vi "DualPump_ExplicitControl.vi"() -> ()   [LabVIEW 2025]
uses:
  <vilib>/Utility/error.llb/DialogType.ctl
  <vilib>/Instr/_visa.llb/VISA Configure Serial Port (Instr).vi
panel:
  out "Arduino Connected":bool
  in  "Arduino Connect Button":bool
  in  "Arduino Fluid Sensor COM Port":refnum<visa-resource-name>
  in  "quit":bool
  in  "Tab Control":enum32{"Control Interface", "Info and Help"}(tab)
  out "Pump #1 Filling":bool
  in  "Pump #1 Partial Fill Amount (µL)":dbl
  in  "Pump #2 Full Fill Button":bool
  in  "Pump #1 Partial Fill Button":bool
  out "Pump #2 Flavor Blasted Amount (µL)":dbl
  out "Pump #1 Flavor Blasted Amount (µL)":dbl
  in  "Pump #2 Start/Stop Button":bool
  in  "Pump #1 COM port":refnum<visa-resource-name>
  in  "Pump #1 flow rate (µL/min)":dbl=2000.0 format="%.3f"
  in  "Pump #2 COM port":refnum<visa-resource-name>
  in  "Pump #2 flow rate (µL/min)":dbl=5000.0 format="%.3f"
  in  "Pump #2 Flavor Blast Amount (µL)":dbl=75.0 format="%.3f"
  in  "Pump #1 syringe volume":dbl(ring)=28.75 items=["100 uL"=1.44, "1 mL"=4.75, "3 mL"=9.8, "5 mL"=11.83, "15 mL"=18.034, "20 mL"=19.304, "50 mL"=28.75]
  in  "Pump #2 syringe volume":dbl(ring)=28.75 items=["100 uL"=1.44, "1 mL"=4.75, "3 mL"=9.8, "5 mL"=11.83, "15 mL"=18.034, "20 mL"=19.304, "50 mL"=28.75]
  out "Pump #2 Flowing":bool
  in  "Pump 1 Connect":bool
  in  "Pump 2 Connect":bool
  out "Pump 2 Connected":bool
  out "Pump 1 Connected":bool
  in  "Pump #1 Flavor Blast Amount (µL)":dbl=200.0
  in  "Pump #1 Flavor Blast Button":bool
  out "Pump #1 Amount Remaining (µL)":dbl
  in  "Pump #1 Start/Stop Button":bool
  out "Pump #1 Flowing":bool
  out "Pump #2 Amount Remaining (µL)":dbl
  in  "Pump #2 Flavor Blast Button":bool
  in  "Pump #2 Partial Fill Button":bool
  in  "Pump #2 Partial Fill Amount (µL)":dbl
  in  "Pump #1 Full Fill Button":bool
  out "Pump #2 Filling":bool
  out "Interface Locked":bool
  # "1. Set Communication"
  # "Pump #1"
  # "Pump #2"
  # "This program is designed to only control the two New Era Syringe Pumps on-site in the Varro laboratory. It can be generalized for other use by adjusting the hard-coded \"firmware\" variables to match any pump.\n\nFull Fill will fill the syringe up to its maximum volume, specified by the chosen syringe volume. Partial Fill will fill the syringe up to the lesser of the chosen volume or the maximum volume.\n\nPumps flow continuously when Start is pressed. The pump will blast a specified amount at its flowrate setpoint when Blast It! is pressed.\n\nFilling and flavor blasting will block the interface, which will be indicated in the upper-right corner."
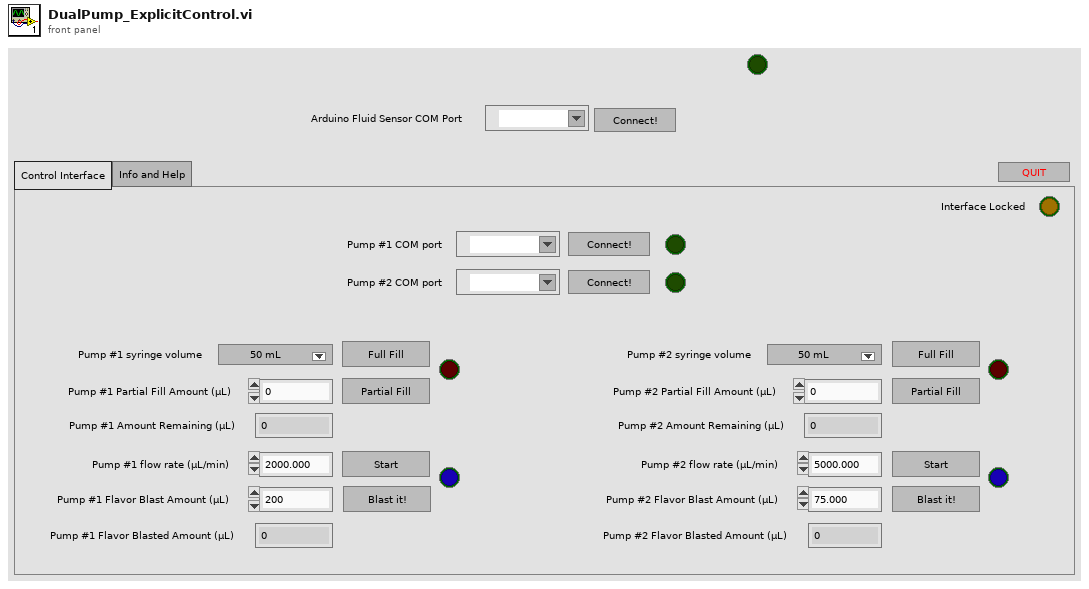
[diagram p1: front panel]
types:
  T1 = cluster{"0=off\n1=on":u16, "Numbers of beeps\n0=continuously":dbl}
  T2 = typedef "DialogType.ctl" = u16
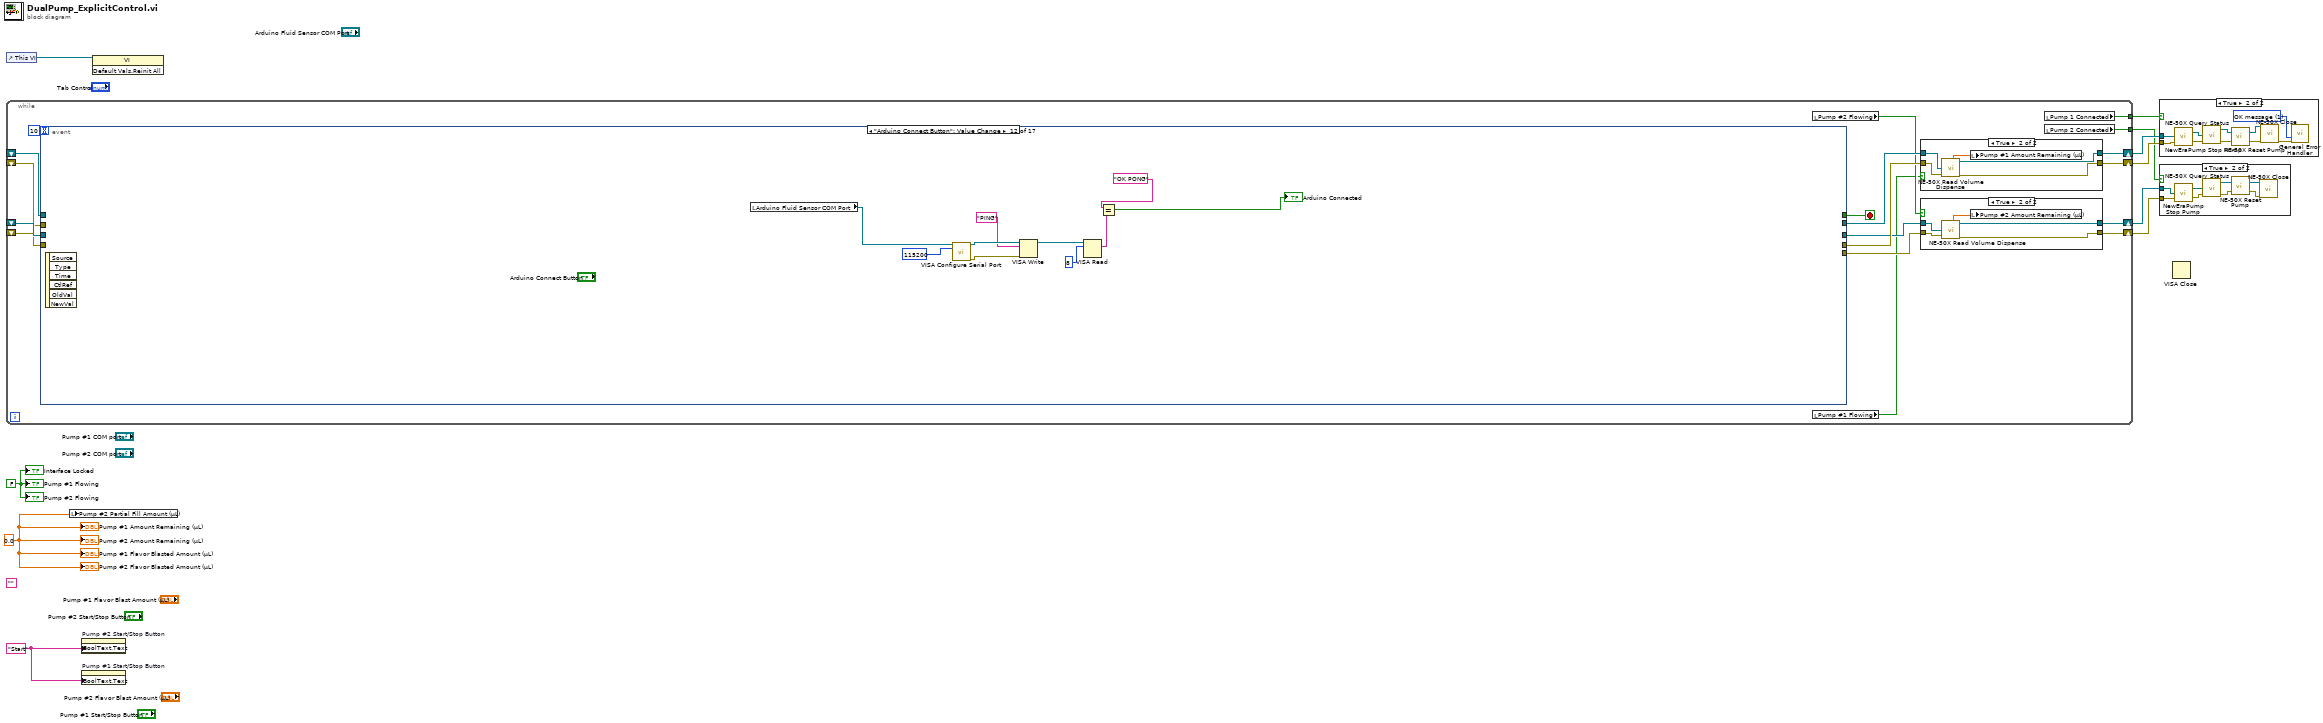
[diagram p0: block diagram]
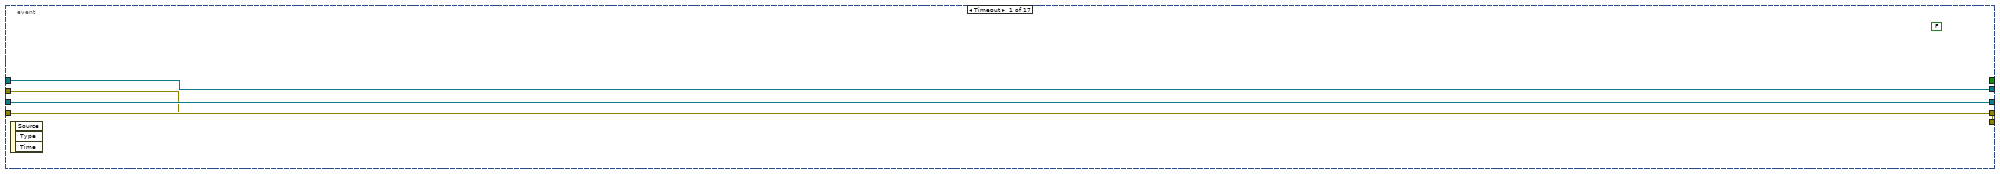
[diagram p6: hidden frame]
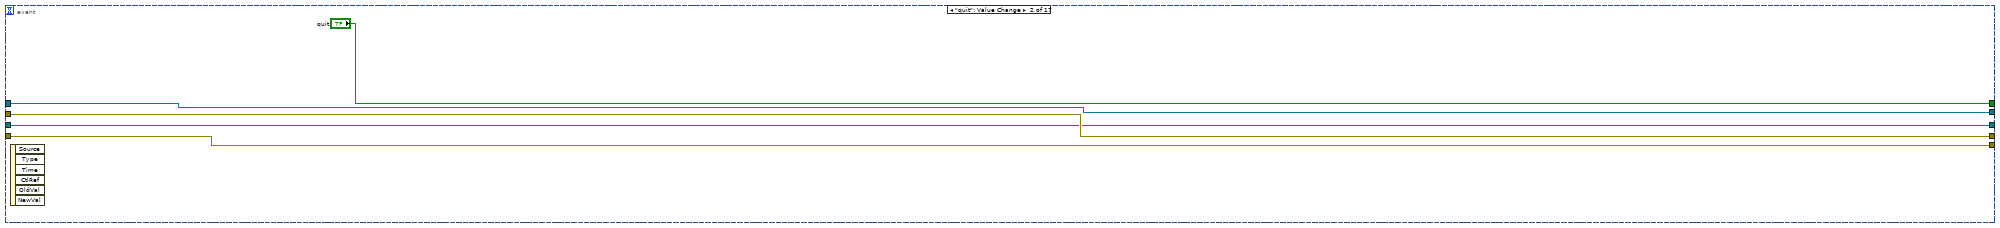
[diagram p7: hidden frame]
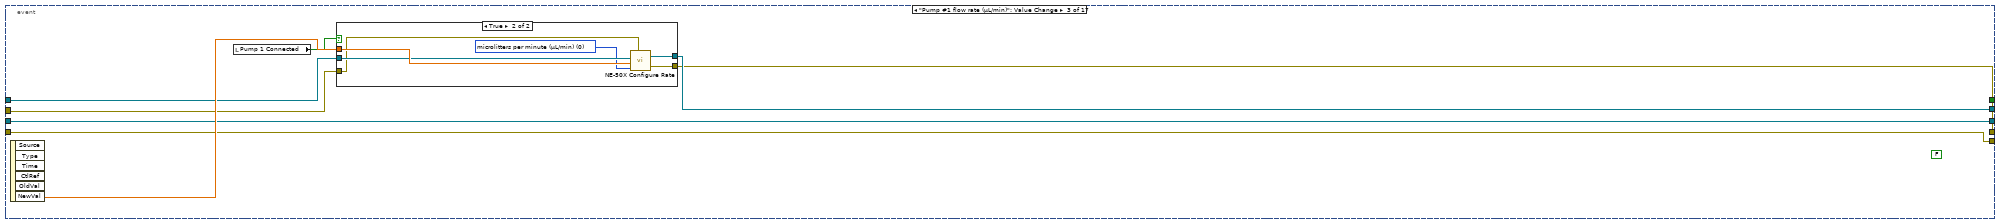
[diagram p8: hidden frame]
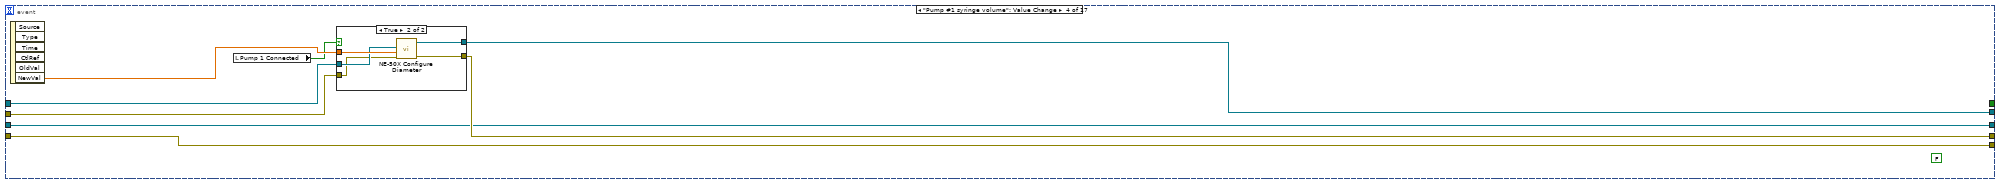
[diagram p10: hidden frame]
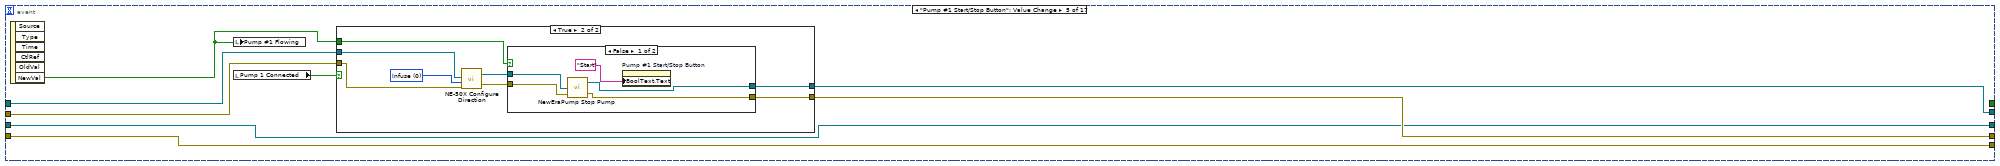
[diagram p12: hidden frame]
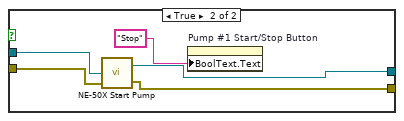
[diagram p14: hidden frame]
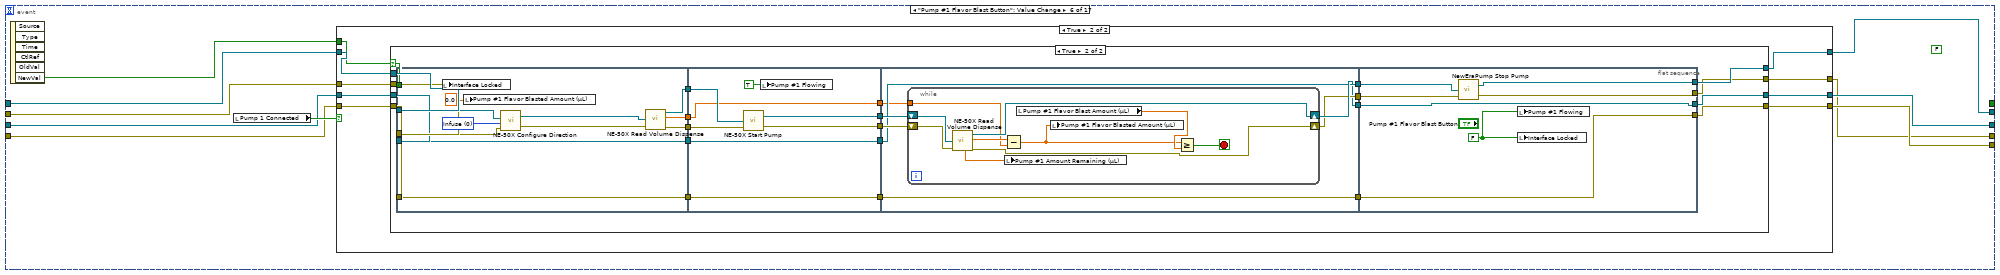
[diagram p15: hidden frame]
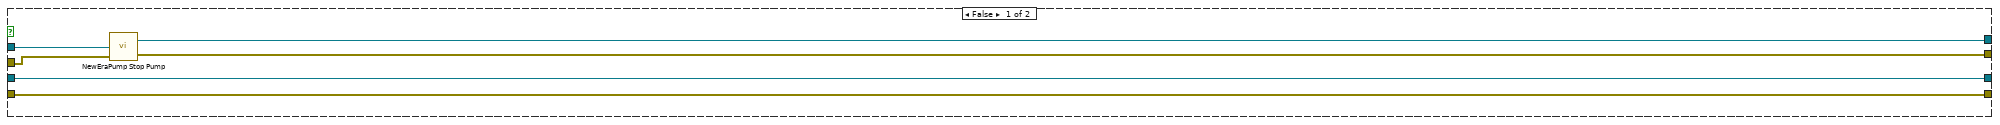
[diagram p17: hidden frame]
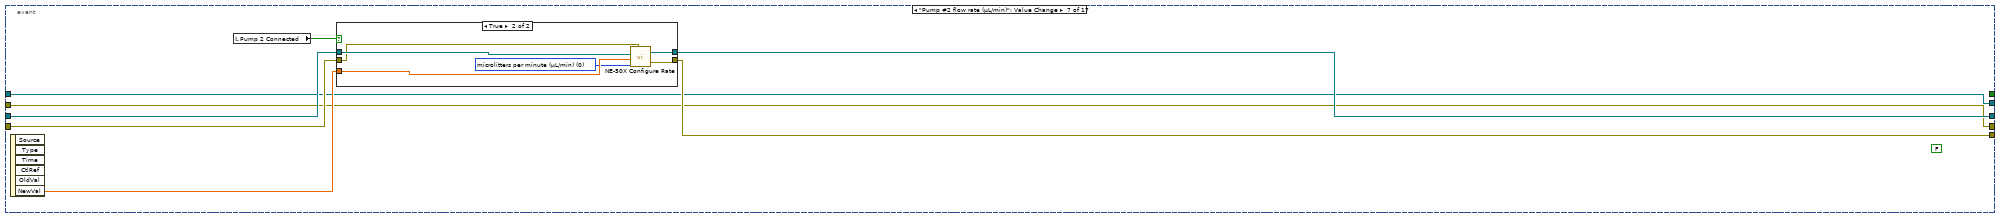
[diagram p18: hidden frame]
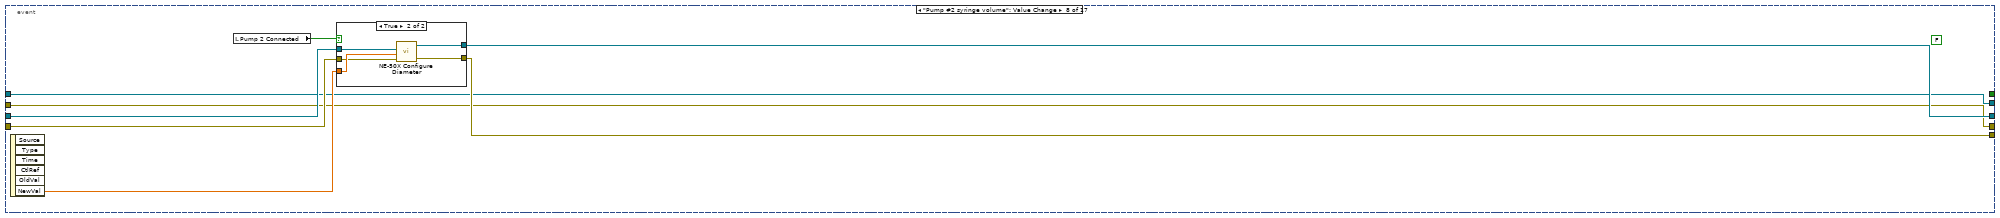
[diagram p20: hidden frame]
diagram:
  w2 = 0.0 ("Pump #1 Flavor Blasted Amount (µL)")
  w1 = FALSE ("0 = Basic")
  w10 = "Start"
  (unwired) ""
  n1 = control-ref of="This VI"() -> (w3:refnum<vi>)
  n2 = while {
    shift-right: [w15] -> w9
    shift-left: _ -> [w28]
    shift-right: [w14] -> w8
    shift-left: _ -> [w27]
    shift-right: [w19] -> w7
    shift-left: _ -> [w25]
    shift-right: [w18] -> w6
    shift-left: _ -> [w26]
    tunnel: [w23] -> w5
    tunnel: [w22] -> w4
    stop <- w11 stop-if-true
    n3 = event shown="[11] \"Arduino Connect Button\": Value Change" {
      selector: _ -> [_ _ _ _ _ _ _ _ _ _ _ _ _ _ _ _ _]
      dyn-events: _ -> [_ _ _ _ _ _ _ _ _ _ _ _ _ _ _ _ _]
      timeout: 10 -> [_ _ _ _ _ _ _ _ _ _ _ _ _ _ _ _ _]
      tunnel: w28 -> [w46 w49 w54 w70 w85 w119 w214 w229 w245 w275 w366 _ _ w452 w538 w619 w722]
      tunnel: w27 -> [w45 w48 w53 w69 w84 w118 w213 w228 w244 w274 w365 _ _ w451 w537 w618 w721]
      tunnel: w25 -> [w44 w51 w58 w74 w90 w117 w209 w225 w239 w269 _ _ w415 w457 _ w622 w718]
      tunnel: w26 -> [w43 w50 w57 w73 w88 w116 w208 w224 w238 w267 _ _ w414 w456 _ w623 w715]
      tunnel: [w46 w49 w54 w70 w85 w113 w212 w227 w241 w273 w366 _ w417 w452 w536 w619 w717] -> w17
      tunnel: [w45 w48 w53 w69 w84 w114 w211 w226 w240 w272 w365 _ w416 w451 w535 w618 w716] -> w16
      tunnel: [w44 w51 w56 w72 w89 w112 w209 w225 w239 w270 w369 _ w415 w454 _ w621 w718] -> w21
      tunnel: [w43 w50 w55 w71 w87 w111 w208 w224 w238 w268 w368 _ w414 w453 _ w620 w715] -> w20
      tunnel: [_ "quit" _ _ _ _ _ _ _ _ _ _ _ _ _ _ _] -> w11
      event Timeout {
        (unwired) FALSE ("quit")
        n4 = event-data() -> ()  [unwired: 1 in, 3 out]
      }
      event "quit": Value Change {
        n5 = event-data() -> ()  [unwired: 1 in, 6 out]
      }
      event "Pump #1 flow rate (µL/min)": Value Change {
        (unwired) FALSE ("quit")
        n6 = event-data() -> ("NewVal"=w59:dbl)  [unwired: 1 in, 5 out]
        n7 = local read "Pump 1 Connected"() -> (w52:bool)
        n8 = case shown="True" w52 {
          tunnel: w59 -> [_ w67]
          tunnel: w58 -> [w61 w66]
          tunnel: w57 -> [w60 w65]
          tunnel: [w61 w63] -> w56
          tunnel: [w60 w62] -> w55
          frame False {
          }
          frame True {
            w64 = 0 items=["microlitters per minute (µL/min)", "microlitters per hour (µL/hr)", "milliliters per minute (mL/min)", "milliliters per hour (µL/hr)"] ("Units")
            n9 = call "NE-50X Configure Rate.vi"("VISA resource name"=w66, "Flow"=w67, "Units"=w64, "error in (no error)"=w65) -> ("VISA resource name out"=w63:refnum<visa-resource-name>, "error out"=w62:errorcluster)  [unwired: 1 in]
          }
        }
      }
      event "Pump #1 syringe volume": Value Change {
        (unwired) FALSE ("quit")
        n10 = event-data() -> ("NewVal"=w75:dbl)  [unwired: 1 in, 5 out]
        n11 = local read "Pump 1 Connected"() -> (w68:bool)
        n12 = case shown="True" w68 {
          tunnel: w75 -> [_ w82]
          tunnel: w74 -> [w76 w81]
          tunnel: w73 -> [w77 w80]
          tunnel: [w76 w79] -> w72
          tunnel: [w77 w78] -> w71
          frame False {
          }
          frame True {
            n13 = call "NE-50X Configure Diameter.vi"("error in (no error)"=w80, "Diameter (19.58 mm)"=w82, "VISA resource name"=w81) -> ("error out"=w78:errorcluster, "VISA resource name out"=w79:refnum<visa-resource-name>)  [unwired: 1 in, 1 out]
          }
        }
      }
      event "Pump #1 Start/Stop Button": Value Change {
        n14 = event-data() -> ("NewVal"=w86:bool)  [unwired: 1 in, 5 out]
        n15 = local write "Pump #1 Flowing"(w86) -> ()
        n16 = local read "Pump 1 Connected"() -> (w83:bool)
        n17 = case shown="True" w83 {
          tunnel: w90 -> [w92 w97]
          tunnel: [w92 w100] -> w89
          tunnel: w88 -> [w91 w96]
          tunnel: [w91 w99] -> w87
          tunnel: w86 -> [_ w98]
          frame False {
          }
          frame True {
            w95 = u16 0 items=["Infuse", "Withdraw"] ("Direction")
            n18 = call "NE-50X Configure Direction.vi"("error in (no error)"=w96, "Direction"=w95, "VISA resource name"=w97) -> ("error out"=w93:errorcluster, "VISA resource name out"=w94:refnum<visa-resource-name>)  [unwired: 1 in]
            n19 = case shown="False" w98 {
              tunnel: [w105 w109] -> w100
              tunnel: [w104 w108] -> w99
              tunnel: w94 -> [w102 w107]
              tunnel: w93 -> [w101 w106]
              frame False {
                n20 = call "NewEraPump Stop Pump.vi"("error in (no error)"=w101, "VISA resource name"=w102) -> ("error out"=w104:errorcluster, "VISA resource name out"=w105:refnum<visa-resource-name>)  [unwired: 1 in]
                n21 = property on="Pump #1 Start/Stop Button" class="Bool"("BoolText.Text"="Start" ("Boolean Text.Text")) -> ()  [unwired: 2 in, 2 out]
              }
              frame True {
                n22 = call "NE-50X Start Pump.vi"("error in (no error)"=w106, "VISA resource name"=w107) -> ("error out"=w108:errorcluster, "VISA resource name out"=w109:refnum<visa-resource-name>)  [unwired: 1 in]
                n23 = property on="Pump #1 Start/Stop Button" class="Bool"("BoolText.Text"="Stop" ("Boolean Text.Text")) -> ()  [unwired: 2 in, 2 out]
              }
            }
          }
        }
      }
      event "Pump #1 Flavor Blast Button": Value Change {
        (unwired) FALSE ("quit")
        n24 = event-data() -> ("NewVal"=w115:bool)  [unwired: 1 in, 5 out]
        n25 = local read "Pump 1 Connected"() -> (w120:bool)
        n26 = case shown="True" w120 {
          tunnel: w117 -> [w122 w133]
          tunnel: w116 -> [w121 w132]
          tunnel: [w122 w131] -> w112
          tunnel: [w121 w130] -> w111
          tunnel: w115 -> [_ w129]
          tunnel: [w124 w128] -> w113
          tunnel: w119 -> [w124 w127]
          tunnel: [w123 w126] -> w114
          tunnel: w118 -> [w123 w125]
          frame False {
          }
          frame True {
            n27 = case shown="True" w129 {
              selector: w129 -> [_ w140]
              tunnel: w133 -> [w139 w162]
              tunnel: [w137 w156] -> w131
              tunnel: w132 -> [w138 w161]
              tunnel: [w136 w155] -> w130
              tunnel: [w135 w154] -> w128
              tunnel: w127 -> [w135 w151]
              tunnel: [w134 w150] -> w126
              tunnel: w125 -> [w134 w147]
              frame False {
                n28 = call "NewEraPump Stop Pump.vi"("error in (no error)"=w138, "VISA resource name"=w139) -> ("error out"=w136:errorcluster, "VISA resource name out"=w137:refnum<visa-resource-name>)  [unwired: 1 in]
              }
              frame True {
                n29 = flat-sequence {
                  tunnel: [w166] -> w146
                  tunnel: [w165] -> w145
                  tunnel: [w174] -> w144
                  tunnel: [w173] -> w143
                  tunnel: [w164] -> w141
                  tunnel: w162 -> [w172]
                  tunnel: w161 -> [w171]
                  tunnel: w151 -> [w174]
                  tunnel: w147 -> [w173]
                  tunnel: w140 -> [w163]
                  tunnel: w146 -> [w182]
                  tunnel: w145 -> [w181]
                  tunnel: [w180] -> w160
                  tunnel: [w179] -> w159
                  tunnel: [w178] -> w152
                  tunnel: w144 -> [w178]
                  tunnel: [w177] -> w148
                  tunnel: w143 -> [w177]
                  tunnel: [w176] -> w142
                  tunnel: w141 -> [w176]
                  tunnel: w160 -> [w189]
                  tunnel: w159 -> [w188]
                  tunnel: [w187] -> w158
                  tunnel: [w186] -> w157
                  tunnel: [w185] -> w153
                  tunnel: w152 -> [w185]
                  tunnel: [w184] -> w149
                  tunnel: w148 -> [w184]
                  tunnel: w142 -> [w183]
                  tunnel: w158 -> [w206]
                  tunnel: w157 -> [w205]
                  tunnel: [w204] -> w156
                  tunnel: [w203] -> w155
                  tunnel: [w202] -> w154
                  tunnel: w153 -> [w202]
                  tunnel: [w201] -> w150
                  tunnel: w149 -> [w201]
                  frame #0 {
                    w170 = u16 0 items=["Infuse", "Withdraw"] ("Direction")
                    n30 = local write "Interface Locked"(w163) -> ()
                    n31 = local write "Pump #1 Flavor Blasted Amount (µL)"(0.0 ("Pump #1 Flavor Blasted Amount (µL)")) -> ()
                    n32 = call "NE-50X Configure Direction.vi"("error in (no error)"=w171, "Direction"=w170, "VISA resource name"=w172) -> ("error out"=w168:errorcluster, "VISA resource name out"=w167:refnum<visa-resource-name>)  [unwired: 1 in]
                    n33 = call "NE-50X Read Volume Dispense.vi"("VISA resource name"=w167, "error in (no error)"=w168) -> ("VISA resource name out"=w166:refnum<visa-resource-name>, "Infused Volume (ul)"=w164:dbl, "error out"=w165:errorcluster)  [unwired: 1 in, 2 out]
                  }
                  frame #1 {
                    n34 = call "NE-50X Start Pump.vi"("error in (no error)"=w181, "VISA resource name"=w182) -> ("error out"=w179:errorcluster, "VISA resource name out"=w180:refnum<visa-resource-name>)  [unwired: 1 in]
                    n35 = local write "Pump #1 Flowing"(TRUE) -> ()
                  }
                  frame #2 {
                    n36 = while {
                      shift-right: [w196] -> w187
                      shift-left: w189 -> [w199]
                      shift-right: [w195] -> w186
                      shift-left: w188 -> [w198]
                      tunnel: w183 -> [w192]
                      stop <- w197 stop-if-true
                      n37 = call "NE-50X Read Volume Dispense.vi"("VISA resource name"=w199, "error in (no error)"=w198) -> ("VISA resource name out"=w196:refnum<visa-resource-name>, "Infused Volume (ul)"=w193:dbl, "error out"=w195:errorcluster, "Amount Remaining (uL)"=w190:dbl)  [unwired: 1 in, 1 out]
                      n38 = Subtract(x=w193, y=w192) -> (x-y=w191:dbl)
                      n39 = local write "Pump #1 Amount Remaining (µL)"(w190) -> ()
                      n40 = local read "Pump #1 Flavor Blast Amount (µL)"() -> (w194:dbl)
                      n41 = local write "Pump #1 Flavor Blasted Amount (µL)"(w191) -> ()
                      n42 = Greater Or Equal?(x=w191, y=w194) -> (x >= y?=w197:bool)
                    }
                  }
                  frame #3 {
                    w200 = FALSE
                    n43 = call "NewEraPump Stop Pump.vi"("error in (no error)"=w205, "VISA resource name"=w206) -> ("error out"=w203:errorcluster, "VISA resource name out"=w204:refnum<visa-resource-name>)  [unwired: 1 in]
                    n44 = local write "Pump #1 Flowing"(w200) -> ()
                    n45 = local write "Interface Locked"(w200) -> ()
                  }
                }
              }
            }
          }
        }
      }
      event "Pump #2 flow rate (µL/min)": Value Change {
        (unwired) FALSE ("quit")
        n46 = event-data() -> ("NewVal"=w210:dbl)  [unwired: 1 in, 5 out]
        n47 = local read "Pump 2 Connected"() -> (w207:bool)
        n48 = case shown="True" w207 {
          tunnel: w214 -> [w216 w222]
          tunnel: w213 -> [w215 w221]
          tunnel: [w216 w220] -> w212
          tunnel: [w215 w219] -> w211
          tunnel: w210 -> [_ w218]
          frame False {
          }
          frame True {
            w217 = 0 items=["microlitters per minute (µL/min)", "microlitters per hour (µL/hr)", "milliliters per minute (mL/min)", "milliliters per hour (µL/hr)"] ("Units")
            n49 = call "NE-50X Configure Rate.vi"("VISA resource name"=w222, "Flow"=w218, "Units"=w217, "error in (no error)"=w221) -> ("VISA resource name out"=w220:refnum<visa-resource-name>, "error out"=w219:errorcluster)  [unwired: 1 in]
          }
        }
      }
      event "Pump #2 syringe volume": Value Change {
        (unwired) FALSE ("quit")
        n50 = event-data() -> ("NewVal"=w230:dbl)  [unwired: 1 in, 5 out]
        n51 = local read "Pump 2 Connected"() -> (w223:bool)
        n52 = case shown="True" w223 {
          tunnel: w230 -> [_ w237]
          tunnel: w229 -> [w231 w236]
          tunnel: w228 -> [w232 w235]
          tunnel: [w231 w234] -> w227
          tunnel: [w232 w233] -> w226
          frame False {
          }
          frame True {
            n53 = call "NE-50X Configure Diameter.vi"("error in (no error)"=w235, "Diameter (19.58 mm)"=w237, "VISA resource name"=w236) -> ("error out"=w233:errorcluster, "VISA resource name out"=w234:refnum<visa-resource-name>)  [unwired: 1 in, 1 out]
          }
        }
      }
      event "Pump #2 Start/Stop Button": Value Change {
        n54 = event-data() -> ("NewVal"=w242:bool)  [unwired: 1 in, 5 out]
        n55 = local write "Pump #2 Flowing"(w242) -> ()
        n56 = local read "Pump 2 Connected"() -> (w243:bool)
        n57 = case shown="True" w243 {
          tunnel: w245 -> [w247 w252]
          tunnel: [w247 w255] -> w241
          tunnel: w244 -> [w246 w250]
          tunnel: [w246 w254] -> w240
          tunnel: w242 -> [_ w253]
          frame False {
          }
          frame True {
            w248 = u16 0 items=["Infuse", "Withdraw"] ("Direction")
            n58 = call "NE-50X Configure Direction.vi"("error in (no error)"=w250, "Direction"=w248, "VISA resource name"=w252) -> ("error out"=w249:errorcluster, "VISA resource name out"=w251:refnum<visa-resource-name>)  [unwired: 1 in]
            n59 = case shown="False" w253 {
              tunnel: w251 -> [w260 w264]
              tunnel: [w258 w263] -> w255
              tunnel: w249 -> [w259 w262]
              tunnel: [w257 w261] -> w254
              frame False {
                n60 = call "NewEraPump Stop Pump.vi"("error in (no error)"=w259, "VISA resource name"=w260) -> ("error out"=w257:errorcluster, "VISA resource name out"=w258:refnum<visa-resource-name>)  [unwired: 1 in]
                n61 = property on="Pump #2 Start/Stop Button" class="Bool"("BoolText.Text"="Start" ("Boolean Text.Text")) -> ()  [unwired: 2 in, 2 out]
              }
              frame True {
                n62 = call "NE-50X Start Pump.vi"("error in (no error)"=w262, "VISA resource name"=w264) -> ("error out"=w261:errorcluster, "VISA resource name out"=w263:refnum<visa-resource-name>)  [unwired: 1 in]
                n63 = property on="Pump #2 Start/Stop Button" class="Bool"("BoolText.Text"="Stop" ("Boolean Text.Text")) -> ()  [unwired: 2 in, 2 out]
              }
            }
          }
        }
      }
      event "Pump #2 Flavor Blast Button": Value Change {
        (unwired) FALSE ("quit")
        n64 = event-data() -> ("NewVal"=w271:bool)  [unwired: 1 in, 5 out]
        n65 = local read "Pump 2 Connected"() -> (w266:bool)
        n66 = case shown="True" w266 {
          tunnel: w275 -> [w277 w288]
          tunnel: w274 -> [w276 w287]
          tunnel: [w277 w286] -> w273
          tunnel: [w276 w285] -> w272
          tunnel: w271 -> [_ w284]
          tunnel: [w279 w283] -> w270
          tunnel: w269 -> [w279 w282]
          tunnel: [w278 w281] -> w268
          tunnel: w267 -> [w278 w280]
          frame False {
          }
          frame True {
            n67 = case shown="True" w284 {
              selector: w284 -> [_ w296]
              tunnel: w288 -> [w295 w318]
              tunnel: [w293 w312] -> w286
              tunnel: w287 -> [w294 w317]
              tunnel: [w292 w311] -> w285
              tunnel: [w290 w310] -> w283
              tunnel: w282 -> [w290 w307]
              tunnel: [w289 w306] -> w281
              tunnel: w280 -> [w289 w303]
              frame False {
                n68 = property on="Pump #2 Flowing" class="Bool (strict)"("BoolText.Text"="Start" ("Boolean Text.Text")) -> ()  [unwired: 2 in, 2 out]
                n69 = call "NewEraPump Stop Pump.vi"("error in (no error)"=w294, "VISA resource name"=w295) -> ("error out"=w292:errorcluster, "VISA resource name out"=w293:refnum<visa-resource-name>)  [unwired: 1 in]
              }
              frame True {
                n70 = flat-sequence {
                  tunnel: [w330] -> w302
                  tunnel: [w329] -> w301
                  tunnel: w318 -> [w327]
                  tunnel: w317 -> [w328]
                  tunnel: w307 -> [w330]
                  tunnel: w303 -> [w329]
                  tunnel: [w323] -> w300
                  tunnel: [w322] -> w299
                  tunnel: [w320] -> w297
                  tunnel: w296 -> [w319]
                  tunnel: [w336] -> w316
                  tunnel: [w335] -> w315
                  tunnel: [w334] -> w308
                  tunnel: w302 -> [w334]
                  tunnel: [w333] -> w304
                  tunnel: w301 -> [w333]
                  tunnel: w300 -> [w338]
                  tunnel: w299 -> [w337]
                  tunnel: [w332] -> w298
                  tunnel: w297 -> [w332]
                  tunnel: w316 -> [w345]
                  tunnel: w315 -> [w344]
                  tunnel: [w343] -> w314
                  tunnel: [w342] -> w313
                  tunnel: [w341] -> w309
                  tunnel: w308 -> [w341]
                  tunnel: [w340] -> w305
                  tunnel: w304 -> [w340]
                  tunnel: w298 -> [w339]
                  tunnel: w314 -> [w362]
                  tunnel: w313 -> [w361]
                  tunnel: [w360] -> w312
                  tunnel: [w359] -> w311
                  tunnel: [w358] -> w310
                  tunnel: w309 -> [w358]
                  tunnel: [w357] -> w306
                  tunnel: w305 -> [w357]
                  frame #0 {
                    w326 = u16 0 items=["Infuse", "Withdraw"] ("Direction")
                    n71 = local write "Interface Locked"(w319) -> ()
                    n72 = local write "Pump #2 Flavor Blasted Amount (µL)"(0.0 ("Pump #2 Flavor Blasted Amount (µL)")) -> ()
                    n73 = call "NE-50X Configure Direction.vi"("error in (no error)"=w328, "Direction"=w326, "VISA resource name"=w327) -> ("error out"=w324:errorcluster, "VISA resource name out"=w325:refnum<visa-resource-name>)  [unwired: 1 in]
                    n74 = call "NE-50X Read Volume Dispense.vi"("VISA resource name"=w325, "error in (no error)"=w324) -> ("VISA resource name out"=w323:refnum<visa-resource-name>, "Infused Volume (ul)"=w320:dbl, "error out"=w322:errorcluster)  [unwired: 1 in, 2 out]
                  }
                  frame #1 {
                    n75 = call "NE-50X Start Pump.vi"("error in (no error)"=w337, "VISA resource name"=w338) -> ("error out"=w335:errorcluster, "VISA resource name out"=w336:refnum<visa-resource-name>)  [unwired: 1 in]
                    n76 = local write "Pump #2 Flowing"(TRUE) -> ()
                  }
                  frame #2 {
                    n77 = while {
                      shift-right: [w351] -> w343
                      shift-left: w345 -> [w355]
                      shift-right: [w350] -> w342
                      shift-left: w344 -> [w354]
                      tunnel: w339 -> [w348]
                      stop <- w353 stop-if-true
                      n78 = call "NE-50X Read Volume Dispense.vi"("VISA resource name"=w355, "error in (no error)"=w354) -> ("VISA resource name out"=w351:refnum<visa-resource-name>, "Infused Volume (ul)"=w349:dbl, "error out"=w350:errorcluster, "Amount Remaining (uL)"=w346:dbl)  [unwired: 1 in, 1 out]
                      n79 = Subtract(x=w349, y=w348) -> (x-y=w347:dbl)
                      n80 = local write "Pump #2 Amount Remaining (µL)"(w346) -> ()
                      n81 = local read "Pump #2 Flavor Blast Amount (µL)"() -> (w352:dbl)
                      n82 = local write "Pump #2 Flavor Blasted Amount (µL)"(w347) -> ()
                      n83 = Greater Or Equal?(x=w347, y=w352) -> (x >= y?=w353:bool)
                    }
                  }
                  frame #3 {
                    w356 = FALSE
                    n84 = call "NewEraPump Stop Pump.vi"("error in (no error)"=w361, "VISA resource name"=w362) -> ("error out"=w359:errorcluster, "VISA resource name out"=w360:refnum<visa-resource-name>)  [unwired: 1 in]
                    n85 = local write "Pump #2 Flowing"(w356) -> ()
                    n86 = local write "Interface Locked"(w356) -> ()
                  }
                }
              }
            }
          }
        }
      }
      event "Pump 1 Connect": Value Change {
        w372 = 0 items=["microlitters per minute (µL/min)", "microlitters per hour (µL/hr)", "milliliters per minute (mL/min)", "milliliters per hour (µL/hr)"] ("Units")
        w363 = u16 0 items=["Infuse", "Withdraw"] ("Direction")
        w377 = 0
        w370 = u16 0 items=["Off", "On"] ("0 = Disabled")
        n87 = event-data() -> ()  [unwired: 1 in, 6 out]
        n88 = local read "Pump #1 COM port"() -> (w367:refnum<visa-resource-name>)
        n89 = call "NE-50X Initialize.vi"("Baud Rate (19200)"=19200, "VISA resource name"=w367) -> ("error out"=w380:errorcluster, "VISA resource name out"=w399:refnum<visa-resource-name>)  [unwired: 1 in]
        n90 = call "NE-50X Read Firmware Version.vi"("error in (no error)"=w380, "VISA resource name"=w399, "Address (0 if unused)"=w377) -> ("error out"=w381:errorcluster, "Version"=w400:string, "VISA resource name out"=w398:refnum<visa-resource-name>)
        n91 = Equal?(x="NE1000V3.934", y=w400) -> (x = y?=→"Pump 1 Connected":bool)
        n92 = call "NE-50X Configure Alarms.vi"("error in (no error)"=w381, "Audible Alarms"=FALSE, "VISA resource name"=w398, "Address (0)"=w377) -> ("error out"=w382:errorcluster, "VISA resource name out"=w397:refnum<visa-resource-name>)
        n93 = call "NE-50X Configure Power Failure Mode.vi"("error in (no error)"=w382, "Power Failure Mode"=w370, "VISA resource name"=w397, "Address (0)"=w377) -> ("error out"=w383:errorcluster, "VISA resource name out"=w396:refnum<visa-resource-name>)
        n94 = call "NE-50X Configure Safe Mode.vi"("error in (no error)"=w383, "Safe Mode"=FALSE ("0 = Basic"), "VISA resource name"=w396, "Address (0)"=w377) -> ("error out"=w387:errorcluster, "VISA resource name out"=w395:refnum<visa-resource-name>)
        n95 = call "NE-50X Clear Volumes.vi"("error in (no error)"=w387, "VISA resource name"=w395, "Address (0)"=w377) -> ("error out"=w379:errorcluster, "VISA resource name out"=w394:refnum<visa-resource-name>)
        n96 = call "NE-50X Configure Diameter.vi"("error in (no error)"=w379, "Diameter (19.58 mm)"="Pump #1 syringe volume", "VISA resource name"=w394, "Address (0)"=w377) -> ("error out"=w388:errorcluster, "VISA resource name out"=w393:refnum<visa-resource-name>)  [unwired: 1 out]
        n97 = call "NE-50X Configure Rate.vi"("Address (0)"=w377, "VISA resource name"=w393, "Flow"="Pump #1 flow rate (µL/min)", "Units"=w372, "error in (no error)"=w388) -> ("VISA resource name out"=w392:refnum<visa-resource-name>, "error out"=w386:errorcluster)
        n98 = call "NE-50X Configure Volume.vi"("error in (no error)"=w386, "Volume"=0.0, "VISA resource name"=w392, "Address (0)"=w377) -> ("error out"=w385:errorcluster, "VISA resource name out"=w391:refnum<visa-resource-name>)
        n99 = call "NE-50X Configure Direction.vi"("error in (no error)"=w385, "Direction"=w363, "VISA resource name"=w391, "Address (0)"=w377) -> ("error out"=w384:errorcluster, "VISA resource name out"=w390:refnum<visa-resource-name>)
        n100 = call "NE-50X Buzzer.vi"("error in (no error)"=w384, "Buzzer"=T1 {"0=off\n1=on"=0, "Numbers of beeps\n0=continuously"=1.0}, "VISA resource name"=w390, "Address (0)"=w377) -> ("error out"=w368:errorcluster, "VISA resource name out"=w369:refnum<visa-resource-name>)
      }
      event "Arduino Connect Button": Value Change {
        n101 = event-data() -> ()  [unwired: 1 in, 6 out]
        n102 = local read "Arduino Fluid Sensor COM Port"() -> (w410:refnum<visa-resource-name>)
        n103 = call-poly "VISA Configure Serial Port"("VISA resource name"=w410, "baud rate (9600)"=u32 115200) -> ("VISA resource name out"=w409:refnum<visa-resource-name>, "error out"=w408:errorcluster)  [unwired: 12 in]
        n104 = VISA Write(VISA resource name=w409, write buffer="PING", error in (no error)=w408) -> (VISA resource name out=w405:refnum<visa-resource-name>)  [unwired: 2 out]
        n105 = VISA Read(VISA resource name=w405, byte count=u32 8) -> (read buffer=w404:string)  [unwired: 1 in, 3 out]
        n106 = Equal?(x="OK PONG", y=w404) -> (x = y?=→"Arduino Connected":bool)
      }
      event "Pump 2 Connect": Value Change {
        (unwired) FALSE ("quit")
        w424 = 0
        w422 = 0 items=["microlitters per minute (µL/min)", "microlitters per hour (µL/hr)", "milliliters per minute (mL/min)", "milliliters per hour (µL/hr)"] ("Units")
        w412 = u16 0 items=["Infuse", "Withdraw"] ("Direction")
        w420 = u16 0 items=["Off", "On"] ("0 = Disabled")
        n107 = event-data() -> ()  [unwired: 1 in, 6 out]
        n108 = local read "Pump #2 COM port"() -> (w427:refnum<visa-resource-name>)
        n109 = call "NE-50X Initialize.vi"("Baud Rate (19200)"=19200, "VISA resource name"=w427) -> ("error out"=w429:errorcluster, "VISA resource name out"=w448:refnum<visa-resource-name>)  [unwired: 1 in]
        n110 = call "NE-50X Read Firmware Version.vi"("error in (no error)"=w429, "VISA resource name"=w448, "Address (0 if unused)"=w424) -> ("error out"=w430:errorcluster, "Version"=w449:string, "VISA resource name out"=w447:refnum<visa-resource-name>)
        n111 = Equal?(x="NE1010V3.934", y=w449) -> (x = y?=→"Pump 2 Connected":bool)
        n112 = call "NE-50X Configure Alarms.vi"("error in (no error)"=w430, "Audible Alarms"=FALSE, "VISA resource name"=w447, "Address (0)"=w424) -> ("error out"=w431:errorcluster, "VISA resource name out"=w446:refnum<visa-resource-name>)
        n113 = call "NE-50X Configure Power Failure Mode.vi"("error in (no error)"=w431, "Power Failure Mode"=w420, "VISA resource name"=w446, "Address (0)"=w424) -> ("error out"=w432:errorcluster, "VISA resource name out"=w445:refnum<visa-resource-name>)
        n114 = call "NE-50X Configure Safe Mode.vi"("error in (no error)"=w432, "Safe Mode"=FALSE ("0 = Basic"), "VISA resource name"=w445, "Address (0)"=w424) -> ("error out"=w436:errorcluster, "VISA resource name out"=w444:refnum<visa-resource-name>)
        n115 = call "NE-50X Clear Volumes.vi"("error in (no error)"=w436, "VISA resource name"=w444, "Address (0)"=w424) -> ("error out"=w428:errorcluster, "VISA resource name out"=w443:refnum<visa-resource-name>)
        n116 = call "NE-50X Configure Diameter.vi"("error in (no error)"=w428, "Diameter (19.58 mm)"="Pump #2 syringe volume", "VISA resource name"=w443, "Address (0)"=w424) -> ("error out"=w437:errorcluster, "VISA resource name out"=w442:refnum<visa-resource-name>)  [unwired: 1 out]
        n117 = call "NE-50X Configure Rate.vi"("Address (0)"=w424, "VISA resource name"=w442, "Flow"="Pump #2 flow rate (µL/min)", "Units"=w422, "error in (no error)"=w437) -> ("VISA resource name out"=w441:refnum<visa-resource-name>, "error out"=w435:errorcluster)
        n118 = call "NE-50X Configure Volume.vi"("error in (no error)"=w435, "Volume"=0.0, "VISA resource name"=w441, "Address (0)"=w424) -> ("error out"=w434:errorcluster, "VISA resource name out"=w440:refnum<visa-resource-name>)
        n119 = call "NE-50X Configure Direction.vi"("error in (no error)"=w434, "Direction"=w412, "VISA resource name"=w440, "Address (0)"=w424) -> ("error out"=w433:errorcluster, "VISA resource name out"=w439:refnum<visa-resource-name>)
        n120 = call "NE-50X Buzzer.vi"("error in (no error)"=w433, "Buzzer"=T1 {"0=off\n1=on"=0, "Numbers of beeps\n0=continuously"=1.0}, "VISA resource name"=w439, "Address (0)"=w424) -> ("error out"=w416:errorcluster, "VISA resource name out"=w417:refnum<visa-resource-name>)
      }
      event "Pump #1 Partial Fill Button": Value Change {
        n121 = event-data() -> ("NewVal"=w455:bool)  [unwired: 1 in, 5 out]
        n122 = local read "Pump 1 Connected"() -> (w458:bool)
        n123 = case shown="True" w458 {
          tunnel: [w460 w465] -> w454
          tunnel: [w459 w464] -> w453
          tunnel: w456 -> [w459 w463]
          tunnel: w457 -> [w460 w462]
          tunnel: w455 -> [_ w461]
          frame False {
          }
          frame True {
            n124 = case shown="True" w461 {
              selector: w461 -> [_ w470]
              tunnel: [w469 w478] -> w465
              tunnel: [w468 w477] -> w464
              tunnel: w463 -> [w466 w474]
              tunnel: w462 -> [w467 w473]
              frame False {
                n125 = call "NewEraPump Stop Pump.vi"("error in (no error)"=w466, "VISA resource name"=w467) -> ("error out"=w468:errorcluster, "VISA resource name out"=w469:refnum<visa-resource-name>)  [unwired: 1 in]
              }
              frame True {
                n126 = flat-sequence {
                  tunnel: [w498] -> w476
                  tunnel: [w497] -> w475
                  tunnel: [w487] -> w471
                  tunnel: w473 -> [w494]
                  tunnel: w474 -> [w492]
                  tunnel: w470 -> [w483]
                  tunnel: w476 -> [w512]
                  tunnel: w475 -> [w511]
                  tunnel: [w510] -> w482
                  tunnel: [w509] -> w481
                  tunnel: [w508] -> w472
                  tunnel: w471 -> [w508]
                  tunnel: w482 -> [w517]
                  tunnel: w481 -> [w516]
                  tunnel: [w515] -> w480
                  tunnel: [w514] -> w479
                  tunnel: w472 -> [w513]
                  tunnel: w480 -> [w531]
                  tunnel: w479 -> [w530]
                  tunnel: [w532] -> w478
                  tunnel: [w534] -> w477
                  frame #0 {
                    w490 = 2 items=["microlitters per minute (µL/min)", "microlitters per hour (µL/hr)", "milliliters per minute (mL/min)", "milliliters per hour (µL/hr)"] ("Units")
                    w496 = u16 1 items=["Infuse", "Withdraw"] ("Direction")
                    n127 = local write "Pump #1 Filling"(w483) -> ()
                    n128 = local write "Interface Locked"(w483) -> ()
                    n129 = property on="Pump #1 syringe volume" class="Ring (strict)"() -> ("RingText.Text"=w486:string)  [unwired: 2 in, 2 out]
                    n130 = case shown="Default" w486 {
                      tunnel: [w499 5.0 ("y") 13.0 ("y") 14.0 ("y") 30.0 ("y")] -> w485
                      tunnel: [w499 5000.0 ("y") 15000.0 ("y") 20000.0 ("y") 50000.0 ("y")] -> w484
                      frame Default {
                        w499 = 0.0 ("y")
                      }
                      frame "5 mL" {
                      }
                      frame "15 mL" {
                      }
                      frame "20 mL" {
                      }
                      frame "50 mL" {
                      }
                    }
                    n131 = Greater Or Equal?(x="Pump #1 Partial Fill Amount (µL)", y=w484) -> (x >= y?=w489:bool)
                    n132 = call "NE-50X Configure Rate.vi"("VISA resource name"=w494, "Flow"=w485, "Units"=w490, "error in (no error)"=w492) -> ("VISA resource name out"=w493:refnum<visa-resource-name>, "error out"=w491:errorcluster)  [unwired: 1 in]
                    n133 = Select(t=w484, s=w489, f="Pump #1 Partial Fill Amount (µL)") -> (s? t:f=w487:dbl)
                    n134 = call "NE-50X Configure Direction.vi"("error in (no error)"=w491, "Direction"=w496, "VISA resource name"=w493, "Address (0)"=0) -> ("error out"=w497:errorcluster, "VISA resource name out"=w498:refnum<visa-resource-name>)
                  }
                  frame #1 {
                    n135 = call "NE-50X Start Pump.vi"("error in (no error)"=w511, "VISA resource name"=w512) -> ("error out"=w509:errorcluster, "VISA resource name out"=w510:refnum<visa-resource-name>)  [unwired: 1 in]
                  }
                  frame #2 {
                    n136 = while {
                      shift-right: [w522] -> w515
                      shift-left: w517 -> [w524]
                      shift-right: [w521] -> w514
                      shift-left: w516 -> [w523]
                      tunnel: w513 -> [w519]
                      stop <- w520 stop-if-true
                      n137 = call "NE-50X Read Volume Dispense.vi"("VISA resource name"=w524, "error in (no error)"=w523) -> ("VISA resource name out"=w522:refnum<visa-resource-name>, "error out"=w521:errorcluster, "Amount Remaining (uL)"=w518:dbl)  [unwired: 1 in, 2 out]
                      n138 = Greater Or Equal?(x=w518, y=w519) -> (x >= y?=w520:bool)
                      n139 = local write "Pump #1 Amount Remaining (µL)"(w518) -> ()
                    }
                  }
                  frame #3 {
                    w533 = 0 items=["microlitters per minute (µL/min)", "microlitters per hour (µL/hr)", "milliliters per minute (mL/min)", "milliliters per hour (µL/hr)"] ("Units")
                    n140 = call "NewEraPump Stop Pump.vi"("error in (no error)"=w530, "VISA resource name"=w531) -> ("error out"=w528:errorcluster, "VISA resource name out"=w529:refnum<visa-resource-name>)  [unwired: 1 in]
                    n141 = Not(x="Pump #1 Partial Fill Button") -> (.not. x?=w525:bool)
                    n142 = local write "Pump #1 Filling"(w525) -> ()
                    n143 = local write "Interface Locked"(w525) -> ()
                    n144 = local read "Pump #1 flow rate (µL/min)"() -> (w527:dbl)
                    n145 = call "NE-50X Configure Rate.vi"("VISA resource name"=w529, "Flow"=w527, "Units"=w533, "error in (no error)"=w528) -> ("VISA resource name out"=w532:refnum<visa-resource-name>, "error out"=w534:errorcluster)  [unwired: 1 in]
                  }
                }
              }
            }
          }
        }
      }
      event "Pump #2 Partial Fill Button": Value Change {
        n146 = event-data() -> ("NewVal"=w539:bool)  [unwired: 1 in, 5 out]
        n147 = local read "Pump 2 Connected"() -> (w540:bool)
        n148 = case shown="True" w540 {
          tunnel: [w542 w547] -> w536
          tunnel: [w541 w546] -> w535
          tunnel: w537 -> [w541 w545]
          tunnel: w538 -> [w542 w544]
          tunnel: w539 -> [_ w543]
          frame False {
          }
          frame True {
            n149 = case shown="True" w543 {
              selector: w543 -> [_ w552]
              tunnel: [w551 w560] -> w547
              tunnel: [w550 w559] -> w546
              tunnel: w545 -> [w548 w556]
              tunnel: w544 -> [w549 w555]
              frame False {
                n150 = call "NewEraPump Stop Pump.vi"("error in (no error)"=w548, "VISA resource name"=w549) -> ("error out"=w550:errorcluster, "VISA resource name out"=w551:refnum<visa-resource-name>)  [unwired: 1 in]
              }
              frame True {
                n151 = flat-sequence {
                  tunnel: [w580] -> w558
                  tunnel: [w579] -> w557
                  tunnel: [w570] -> w553
                  tunnel: w555 -> [w576]
                  tunnel: w556 -> [w574]
                  tunnel: w552 -> [w565]
                  tunnel: w558 -> [w594]
                  tunnel: w557 -> [w593]
                  tunnel: [w592] -> w564
                  tunnel: [w591] -> w563
                  tunnel: [w590] -> w554
                  tunnel: w553 -> [w590]
                  tunnel: w564 -> [w599]
                  tunnel: w563 -> [w598]
                  tunnel: [w597] -> w562
                  tunnel: [w596] -> w561
                  tunnel: w554 -> [w595]
                  tunnel: w562 -> [w613]
                  tunnel: w561 -> [w612]
                  tunnel: [w614] -> w560
                  tunnel: [w616] -> w559
                  frame #0 {
                    w572 = 2 items=["microlitters per minute (µL/min)", "microlitters per hour (µL/hr)", "milliliters per minute (mL/min)", "milliliters per hour (µL/hr)"] ("Units")
                    w578 = u16 1 items=["Infuse", "Withdraw"] ("Direction")
                    n152 = local write "Pump #2 Filling"(w565) -> ()
                    n153 = local write "Interface Locked"(w565) -> ()
                    n154 = property on="Pump #2 syringe volume" class="Ring (strict)"() -> ("RingText.Text"=w568:string)  [unwired: 2 in, 2 out]
                    n155 = case shown="Default" w568 {
                      tunnel: [w581 5.0 ("y") 13.0 ("y") 14.0 ("y") 30.0 ("y")] -> w567
                      tunnel: [w581 5000.0 ("y") 15000.0 ("y") 20000.0 ("y") 50000.0 ("y")] -> w566
                      frame Default {
                        w581 = 0.0 ("y")
                      }
                      frame "5 mL" {
                      }
                      frame "15 mL" {
                      }
                      frame "20 mL" {
                      }
                      frame "50 mL" {
                      }
                    }
                    n156 = Greater Or Equal?(x="Pump #2 Partial Fill Amount (µL)", y=w566) -> (x >= y?=w571:bool)
                    n157 = call "NE-50X Configure Rate.vi"("VISA resource name"=w576, "Flow"=w567, "Units"=w572, "error in (no error)"=w574) -> ("VISA resource name out"=w575:refnum<visa-resource-name>, "error out"=w573:errorcluster)  [unwired: 1 in]
                    n158 = Select(t=w566, s=w571, f="Pump #2 Partial Fill Amount (µL)") -> (s? t:f=w570:dbl)
                    n159 = call "NE-50X Configure Direction.vi"("error in (no error)"=w573, "Direction"=w578, "VISA resource name"=w575, "Address (0)"=0) -> ("error out"=w579:errorcluster, "VISA resource name out"=w580:refnum<visa-resource-name>)
                  }
                  frame #1 {
                    n160 = call "NE-50X Start Pump.vi"("error in (no error)"=w593, "VISA resource name"=w594) -> ("error out"=w591:errorcluster, "VISA resource name out"=w592:refnum<visa-resource-name>)  [unwired: 1 in]
                  }
                  frame #2 {
                    n161 = while {
                      shift-right: [w604] -> w597
                      shift-left: w599 -> [w606]
                      shift-right: [w603] -> w596
                      shift-left: w598 -> [w605]
                      tunnel: w595 -> [w601]
                      stop <- w602 stop-if-true
                      n162 = call "NE-50X Read Volume Dispense.vi"("VISA resource name"=w606, "error in (no error)"=w605) -> ("VISA resource name out"=w604:refnum<visa-resource-name>, "error out"=w603:errorcluster, "Amount Remaining (uL)"=w600:dbl)  [unwired: 1 in, 2 out]
                      n163 = Greater Or Equal?(x=w600, y=w601) -> (x >= y?=w602:bool)
                      n164 = local write "Pump #2 Amount Remaining (µL)"(w600) -> ()
                    }
                  }
                  frame #3 {
                    w615 = 0 items=["microlitters per minute (µL/min)", "microlitters per hour (µL/hr)", "milliliters per minute (mL/min)", "milliliters per hour (µL/hr)"] ("Units")
                    n165 = call "NewEraPump Stop Pump.vi"("error in (no error)"=w612, "VISA resource name"=w613) -> ("error out"=w610:errorcluster, "VISA resource name out"=w611:refnum<visa-resource-name>)  [unwired: 1 in]
                    n166 = Not(x="Pump #2 Partial Fill Button") -> (.not. x?=w607:bool)
                    n167 = local write "Pump #2 Filling"(w607) -> ()
                    n168 = local write "Interface Locked"(w607) -> ()
                    n169 = local read "Pump #2 flow rate (µL/min)"() -> (w609:dbl)
                    n170 = call "NE-50X Configure Rate.vi"("VISA resource name"=w611, "Flow"=w609, "Units"=w615, "error in (no error)"=w610) -> ("VISA resource name out"=w614:refnum<visa-resource-name>, "error out"=w616:errorcluster)  [unwired: 1 in]
                  }
                }
              }
            }
          }
        }
      }
      event "Pump #1 Full Fill Button": Value Change {
        n171 = event-data() -> ("NewVal"=w617:bool)  [unwired: 1 in, 5 out]
        n172 = local read "Pump 1 Connected"() -> (w624:bool)
        n173 = case shown="True" w624 {
          tunnel: [w626 w631] -> w621
          tunnel: [w625 w630] -> w620
          tunnel: w623 -> [w625 w629]
          tunnel: w622 -> [w626 w628]
          tunnel: w617 -> [_ w627]
          frame False {
          }
          frame True {
            n174 = case shown="True" w627 {
              selector: w627 -> [_ w636]
              tunnel: [w635 w644] -> w631
              tunnel: [w634 w643] -> w630
              tunnel: w629 -> [w632 w640]
              tunnel: w628 -> [w633 w639]
              frame False {
                n175 = call "NewEraPump Stop Pump.vi"("error in (no error)"=w632, "VISA resource name"=w633) -> ("error out"=w634:errorcluster, "VISA resource name out"=w635:refnum<visa-resource-name>)  [unwired: 1 in]
              }
              frame True {
                n176 = flat-sequence {
                  tunnel: [w660] -> w642
                  tunnel: [w659] -> w641
                  tunnel: w639 -> [w656]
                  tunnel: w640 -> [w654]
                  tunnel: [w651] -> w637
                  tunnel: w636 -> [w649]
                  tunnel: w642 -> [w670]
                  tunnel: w641 -> [w669]
                  tunnel: [w668] -> w648
                  tunnel: [w667] -> w647
                  tunnel: [w666] -> w638
                  tunnel: w637 -> [w666]
                  tunnel: w648 -> [w675]
                  tunnel: w647 -> [w674]
                  tunnel: [w673] -> w646
                  tunnel: [w672] -> w645
                  tunnel: w638 -> [w671]
                  tunnel: w646 -> [w711]
                  tunnel: w645 -> [w709]
                  tunnel: [w712] -> w644
                  tunnel: [w714] -> w643
                  frame #0 {
                    w652 = 2 items=["microlitters per minute (µL/min)", "microlitters per hour (µL/hr)", "milliliters per minute (mL/min)", "milliliters per hour (µL/hr)"] ("Units")
                    w658 = u16 1 items=["Infuse", "Withdraw"] ("Direction")
                    n177 = local write "Interface Locked"(w649) -> ()
                    n178 = property on="Pump #1 syringe volume" class="Ring (strict)"() -> ("RingText.Text"=w651:string)  [unwired: 2 in, 2 out]
                    n179 = case shown="\"50 mL\"" w651 {
                      tunnel: [0.0 ("y") 5.0 ("y") 13.0 ("y") 14.0 ("y") 30.0 ("y")] -> w650
                      frame Default {
                      }
                      frame "5 mL" {
                      }
                      frame "15 mL" {
                      }
                      frame "20 mL" {
                      }
                      frame "50 mL" {
                      }
                    }
                    n180 = call "NE-50X Configure Rate.vi"("VISA resource name"=w656, "Flow"=w650, "Units"=w652, "error in (no error)"=w654) -> ("VISA resource name out"=w655:refnum<visa-resource-name>, "error out"=w653:errorcluster)  [unwired: 1 in]
                    n181 = call "NE-50X Configure Direction.vi"("error in (no error)"=w653, "Direction"=w658, "VISA resource name"=w655, "Address (0)"=0) -> ("error out"=w659:errorcluster, "VISA resource name out"=w660:refnum<visa-resource-name>)
                    "Pump #1 Filling" <- w649
                  }
                  frame #1 {
                    n182 = call "NE-50X Start Pump.vi"("error in (no error)"=w669, "VISA resource name"=w670) -> ("error out"=w667:errorcluster, "VISA resource name out"=w668:refnum<visa-resource-name>)  [unwired: 1 in]
                  }
                  frame #2 {
                    n183 = while {
                      shift-right: [w679] -> w673
                      shift-left: w675 -> [w682]
                      shift-right: [w678] -> w672
                      shift-left: w674 -> [w681]
                      tunnel: w671 -> [w677]
                      stop <- w680 stop-if-true
                      n184 = call "NE-50X Read Volume Dispense.vi"("VISA resource name"=w682, "error in (no error)"=w681) -> ("VISA resource name out"=w679:refnum<visa-resource-name>, "error out"=w678:errorcluster, "Amount Remaining (uL)"=w676:dbl)  [unwired: 1 in, 2 out]
                      n185 = case shown="\"5 mL\"" w677 {
                        tunnel: [TRUE w684 w688 w691 w693 w696 w699 w702] -> w680
                        tunnel: w676 -> [_ w685 w687 w690 w694 w697 w700 w703]
                        frame Default {
                        }
                        frame "100 uL" {
                          n186 = Greater Or Equal?(x=w685, y=100.0) -> (x >= y?=w684:bool)
                        }
                        frame "1 mL" {
                          n187 = Greater Or Equal?(x=w687, y=1000.0) -> (x >= y?=w688:bool)
                        }
                        frame "3 mL" {
                          n188 = Greater Or Equal?(x=w690, y=3000.0) -> (x >= y?=w691:bool)
                        }
                        frame "5 mL" {
                          n189 = Greater Or Equal?(x=w694, y=5000.0) -> (x >= y?=w693:bool)
                        }
                        frame "15 mL" {
                          n190 = Greater Or Equal?(x=w697, y=15000.0) -> (x >= y?=w696:bool)
                        }
                        frame "20 mL" {
                          n191 = Greater Or Equal?(x=w700, y=20000.0) -> (x >= y?=w699:bool)
                        }
                        frame "50 mL" {
                          n192 = Greater Or Equal?(x=w703, y=50000.0) -> (x >= y?=w702:bool)
                        }
                      }
                      n193 = local write "Pump #1 Amount Remaining (µL)"(w676) -> ()
                    }
                  }
                  frame #3 {
                    w713 = 0 items=["microlitters per minute (µL/min)", "microlitters per hour (µL/hr)", "milliliters per minute (mL/min)", "milliliters per hour (µL/hr)"] ("Units")
                    n194 = call "NewEraPump Stop Pump.vi"("error in (no error)"=w709, "VISA resource name"=w711) -> ("error out"=w708:errorcluster, "VISA resource name out"=w710:refnum<visa-resource-name>)  [unwired: 1 in]
                    n195 = Not(x="Pump #1 Full Fill Button") -> (.not. x?=w705:bool)
                    n196 = local read "Pump #1 flow rate (µL/min)"() -> (w707:dbl)
                    n197 = local write "Pump #1 Filling"(w705) -> ()
                    n198 = local write "Interface Locked"(w705) -> ()
                    n199 = call "NE-50X Configure Rate.vi"("VISA resource name"=w710, "Flow"=w707, "Units"=w713, "error in (no error)"=w708) -> ("VISA resource name out"=w712:refnum<visa-resource-name>, "error out"=w714:errorcluster)  [unwired: 1 in]
                  }
                }
              }
            }
          }
        }
      }
      event "Pump #2 Full Fill Button": Value Change {
        n200 = event-data() -> ("NewVal"=w720:bool)  [unwired: 1 in, 5 out]
        n201 = local read "Pump 2 Connected"() -> (w719:bool)
        n202 = case shown="True" w719 {
          tunnel: [w724 w729] -> w717
          tunnel: [w723 w728] -> w716
          tunnel: w721 -> [w723 w727]
          tunnel: w722 -> [w724 w726]
          tunnel: w720 -> [_ w725]
          frame False {
          }
          frame True {
            n203 = case shown="True" w725 {
              selector: w725 -> [_ w734]
              tunnel: [w733 w742] -> w729
              tunnel: [w732 w741] -> w728
              tunnel: w727 -> [w730 w738]
              tunnel: w726 -> [w731 w737]
              frame False {
                n204 = call "NewEraPump Stop Pump.vi"("error in (no error)"=w730, "VISA resource name"=w731) -> ("error out"=w732:errorcluster, "VISA resource name out"=w733:refnum<visa-resource-name>)  [unwired: 1 in]
              }
              frame True {
                n205 = flat-sequence {
                  tunnel: [w758] -> w740
                  tunnel: [w757] -> w739
                  tunnel: w737 -> [w753]
                  tunnel: w738 -> [w751]
                  tunnel: [w748] -> w735
                  tunnel: w734 -> [w747]
                  tunnel: w740 -> [w768]
                  tunnel: w739 -> [w767]
                  tunnel: [w766] -> w746
                  tunnel: [w765] -> w745
                  tunnel: [w764] -> w736
                  tunnel: w735 -> [w764]
                  tunnel: w746 -> [w773]
                  tunnel: w745 -> [w772]
                  tunnel: [w771] -> w744
                  tunnel: [w770] -> w743
                  tunnel: w736 -> [w769]
                  tunnel: w744 -> [w809]
                  tunnel: w743 -> [w807]
                  tunnel: [w810] -> w742
                  tunnel: [w812] -> w741
                  frame #0 {
                    w754 = 2 items=["microlitters per minute (µL/min)", "microlitters per hour (µL/hr)", "milliliters per minute (mL/min)", "milliliters per hour (µL/hr)"] ("Units")
                    w756 = u16 1 items=["Infuse", "Withdraw"] ("Direction")
                    n206 = local write "Interface Locked"(w747) -> ()
                    n207 = property on="Pump #2 syringe volume" class="Ring (strict)"() -> ("RingText.Text"=w748:string)  [unwired: 2 in, 2 out]
                    n208 = case shown="\"50 mL\"" w748 {
                      tunnel: [0.0 ("y") 5.0 ("y") 13.0 ("y") 14.0 ("y") 30.0 ("y")] -> w749
                      frame Default {
                      }
                      frame "5 mL" {
                      }
                      frame "15 mL" {
                      }
                      frame "20 mL" {
                      }
                      frame "50 mL" {
                      }
                    }
                    n209 = call "NE-50X Configure Rate.vi"("VISA resource name"=w753, "Flow"=w749, "Units"=w754, "error in (no error)"=w751) -> ("VISA resource name out"=w752:refnum<visa-resource-name>, "error out"=w750:errorcluster)  [unwired: 1 in]
                    n210 = call "NE-50X Configure Direction.vi"("error in (no error)"=w750, "Direction"=w756, "VISA resource name"=w752, "Address (0)"=0) -> ("error out"=w757:errorcluster, "VISA resource name out"=w758:refnum<visa-resource-name>)
                    "Pump #2 Filling" <- w747
                  }
                  frame #1 {
                    n211 = call "NE-50X Start Pump.vi"("error in (no error)"=w767, "VISA resource name"=w768) -> ("error out"=w765:errorcluster, "VISA resource name out"=w766:refnum<visa-resource-name>)  [unwired: 1 in]
                  }
                  frame #2 {
                    n212 = while {
                      shift-right: [w778] -> w771
                      shift-left: w773 -> [w780]
                      shift-right: [w777] -> w770
                      shift-left: w772 -> [w779]
                      tunnel: w769 -> [w776]
                      stop <- w774 stop-if-true
                      n213 = call "NE-50X Read Volume Dispense.vi"("VISA resource name"=w780, "error in (no error)"=w779) -> ("VISA resource name out"=w778:refnum<visa-resource-name>, "error out"=w777:errorcluster, "Amount Remaining (uL)"=w775:dbl)  [unwired: 1 in, 2 out]
                      n214 = case shown="\"5 mL\"" w776 {
                        tunnel: [TRUE w782 w786 w789 w791 w794 w797 w800] -> w774
                        tunnel: w775 -> [_ w783 w785 w788 w792 w795 w798 w801]
                        frame Default {
                        }
                        frame "100 uL" {
                          n215 = Greater Or Equal?(x=w783, y=100.0) -> (x >= y?=w782:bool)
                        }
                        frame "1 mL" {
                          n216 = Greater Or Equal?(x=w785, y=1000.0) -> (x >= y?=w786:bool)
                        }
                        frame "3 mL" {
                          n217 = Greater Or Equal?(x=w788, y=3000.0) -> (x >= y?=w789:bool)
                        }
                        frame "5 mL" {
                          n218 = Greater Or Equal?(x=w792, y=5000.0) -> (x >= y?=w791:bool)
                        }
                        frame "15 mL" {
                          n219 = Greater Or Equal?(x=w795, y=15000.0) -> (x >= y?=w794:bool)
                        }
                        frame "20 mL" {
                          n220 = Greater Or Equal?(x=w798, y=20000.0) -> (x >= y?=w797:bool)
                        }
                        frame "50 mL" {
                          n221 = Greater Or Equal?(x=w801, y=50000.0) -> (x >= y?=w800:bool)
                        }
                      }
                      n222 = local write "Pump #2 Amount Remaining (µL)"(w775) -> ()
                    }
                  }
                  frame #3 {
                    w811 = 0 items=["microlitters per minute (µL/min)", "microlitters per hour (µL/hr)", "milliliters per minute (mL/min)", "milliliters per hour (µL/hr)"] ("Units")
                    n223 = call "NewEraPump Stop Pump.vi"("error in (no error)"=w807, "VISA resource name"=w809) -> ("error out"=w806:errorcluster, "VISA resource name out"=w808:refnum<visa-resource-name>)  [unwired: 1 in]
                    n224 = Not(x="Pump #2 Full Fill Button") -> (.not. x?=w803:bool)
                    n225 = local read "Pump #2 flow rate (µL/min)"() -> (w805:dbl)
                    n226 = local write "Pump #2 Filling"(w803) -> ()
                    n227 = local write "Interface Locked"(w803) -> ()
                    n228 = call "NE-50X Configure Rate.vi"("VISA resource name"=w808, "Flow"=w805, "Units"=w811, "error in (no error)"=w806) -> ("VISA resource name out"=w810:refnum<visa-resource-name>, "error out"=w812:errorcluster)  [unwired: 1 in]
                  }
                }
              }
            }
          }
        }
      }
    }
    n229 = local read "Pump #2 Flowing"() -> (w13:bool)
    n230 = local read "Pump #1 Flowing"() -> (w12:bool)
    n231 = case shown="True" w12 {
      tunnel: w21 -> [w37 w42]
      tunnel: w20 -> [w36 w41]
      tunnel: [w37 w40] -> w19
      tunnel: [w36 w39] -> w18
      frame False {
      }
      frame True {
        n232 = call "NE-50X Read Volume Dispense.vi"("VISA resource name"=w42, "error in (no error)"=w41) -> ("VISA resource name out"=w40:refnum<visa-resource-name>, "error out"=w39:errorcluster, "Amount Remaining (uL)"=w38:dbl)  [unwired: 1 in, 2 out]
        n233 = local write "Pump #1 Amount Remaining (µL)"(w38) -> ()
      }
    }
    n234 = case shown="True" w13 {
      tunnel: w17 -> [w30 w35]
      tunnel: w16 -> [w29 w34]
      tunnel: [w30 w33] -> w15
      tunnel: [w29 w32] -> w14
      frame False {
      }
      frame True {
        n235 = call "NE-50X Read Volume Dispense.vi"("VISA resource name"=w35, "error in (no error)"=w34) -> ("VISA resource name out"=w33:refnum<visa-resource-name>, "error out"=w32:errorcluster, "Amount Remaining (uL)"=w31:dbl)  [unwired: 1 in, 2 out]
        n236 = local write "Pump #2 Amount Remaining (µL)"(w31) -> ()
      }
    }
    n237 = local read "Pump 1 Connected"() -> (w22:bool)
    n238 = local read "Pump 2 Connected"() -> (w23:bool)
  }
  n239 = local write "Pump #2 Partial Fill Amount (µL)"(w2) -> ()
  n240 = property on="Pump #2 Start/Stop Button" class="Bool"("BoolText.Text"=w10) -> ()  [unwired: 2 in, 2 out]
  n241 = property on="Pump #1 Start/Stop Button" class="Bool"("BoolText.Text"=w10) -> ()  [unwired: 2 in, 2 out]
  n242 = invoke class="VI" method="Default Vals.Reinit All"(reference=w3) -> ()  [unwired: 2 in, 3 out]
  n243 = case shown="True" w4 {
    tunnel: w7 -> [_ w814]
    tunnel: w6 -> [_ w813]
    frame False {
    }
    frame True {
      w817 = T2 1 items=["no dialog", "OK message", "continue or stop message", "OK message + warnings", "continue/stop + warnings"] ("type of dialog (OK msg:1)")
      n244 = call "NewEraPump Stop Pump.vi"("error in (no error)"=w813, "VISA resource name"=w814) -> ("error out"=w816:errorcluster, "VISA resource name out"=w815:refnum<visa-resource-name>)  [unwired: 1 in]
      n245 = call "NE-50X Query Status.vi"("error in (no error)"=w816, "VISA resource name"=w815) -> ("error out"=w820:errorcluster, "VISA resource name out"=w821:refnum<visa-resource-name>)  [unwired: 1 in, 1 out]
      n246 = call "NE-50X Reset Pump.vi"("error in (no error)"=w820, "VISA resource name"=w821) -> ("error out"=w819:errorcluster, "VISA resource name out"=w822:refnum<visa-resource-name>)
      n247 = call "NE-50X Close.vi"("VISA resource name"=w822, "error in (no error)"=w819) -> ("error out"=w818:errorcluster)  [unwired: 13 in]
      n248 = call <vilib>:"General Error Handler.vi"("type of dialog (OK msg:1)"=w817, "error in (no error)"=w818) -> ()  [unwired: 9 in, 5 out]
    }
  }
  n249 = case shown="True" w5 {
    tunnel: w9 -> [_ w824]
    tunnel: w8 -> [_ w823]
    frame False {
    }
    frame True {
      n250 = call "NewEraPump Stop Pump.vi"("error in (no error)"=w823, "VISA resource name"=w824) -> ("error out"=w825:errorcluster, "VISA resource name out"=w826:refnum<visa-resource-name>)  [unwired: 1 in]
      n251 = call "NE-50X Query Status.vi"("error in (no error)"=w825, "VISA resource name"=w826) -> ("error out"=w828:errorcluster, "VISA resource name out"=w829:refnum<visa-resource-name>)  [unwired: 1 in, 1 out]
      n252 = call "NE-50X Reset Pump.vi"("error in (no error)"=w828, "VISA resource name"=w829) -> ("error out"=w827:errorcluster, "VISA resource name out"=w830:refnum<visa-resource-name>)
      n253 = call "NE-50X Close.vi"("VISA resource name"=w830, "error in (no error)"=w827) -> ()  [unwired: 13 in, 1 out]
    }
  }
  n254 = VISA Close() -> ()  [unwired: 2 in, 1 out]
  "Pump #2 Flowing" <- w1
  "Pump #1 Flowing" <- w1
  "Pump #1 Flavor Blasted Amount (µL)" <- w2
  "Pump #1 Amount Remaining (µL)" <- w2
  "Pump #2 Amount Remaining (µL)" <- w2
  "Pump #2 Flavor Blasted Amount (µL)" <- w2
  "Interface Locked" <- w1
